vi "[ce] Find All Minima and Maxima of f(x).vi"(5 "accuracy":dbl=1e-08 format="%.2e", 6 "parameters":cluster{"name":string, "value":dbl}[](array[cluster]) {"value" format="%.2f"}, 7 "# points":u32=1000, 8 "error in":errorcluster, 9 "formula info":cluster{"formula":string, "x-variable":string}, 10 "end":dbl=1.0 format="%.2f", 11 "start":dbl format="%.2f") -> (0 "error out":errorcluster, 1 "ticks":u32, 2 "minima":cluster{"x":dbl[], "f(x)":dbl[]} {"f(x)" format="%.2f"; "x" format="%.2f"}, 3 "maxima":cluster{"x":dbl[], "f(x)":dbl[]} {"f(x)" format="%.2f"; "x" format="%.2f"})   [LabVIEW 2021]
doc: "The VI searches for all local minima and maxima of a 1D function in the specified interval. In addition, the VI allows specifying additional parameters and evaluating them in formula.\n\n::: CalcExpress Toolkit :::\nCopyright (c) 2000-2026 Konstantin Shifershteyn. All rights reserved."
panel:
  # "Example:\n\n accuracy: 1E-8 \n start: 0.0\n end: 1.0\n formula: x*x+sin(x)-1\n x-variable: x"
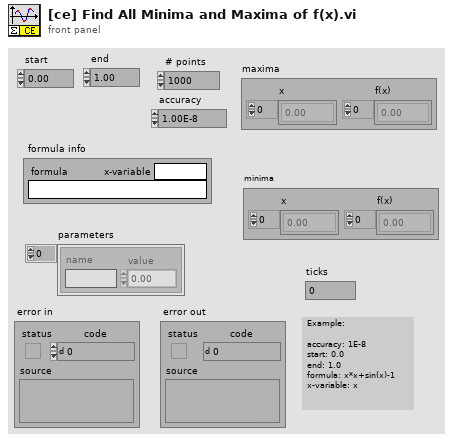
[diagram p1: front panel]
types:
  T1 = typedef "VarMan Variable Context Handle.ctl" = i32
  T2 = enum16{"create", "destroy", "set value", "get value"}
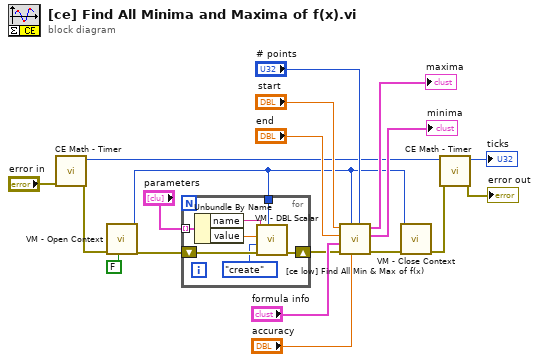
[diagram p0: block diagram]
diagram:
  n1 = call "CE Math - Timer.vi"("error in (no error)"="error in") -> ("error out"=w18:errorcluster, "ticks out"=w6:u32)  [unwired: 7 in]
  n2 = call "VM - Open Context.vi"("close loose contexts (F)"=FALSE ("close loose contexts (T)"), "error in"=w18) -> ("error out"=w4:errorcluster, "VC Handle out"=w2:T1)  [unwired: 7 in, 1 out]
  n3 = for {
    shift-right: [w23] -> w5
    shift-left: w4 -> [w24]
    tunnel: "parameters" -> [w21] mode=indexing
    tunnel: w2 -> [w20]
    n4 = Unbundle By Name(w21) -> ("name"=w25:string, "value"=w26:dbl)
    n5 = call "VM - DBL Scalar.vi"("VC Handle"=w20, "error in"=w24, "cmd"=T2."create", "value in"=w26, "name_spec"=w25) -> ("error out"=w23:errorcluster)  [unwired: 1 in, 5 out]
  }
  n6 = call "[ce low] Find All Min & Max of f(x).vi"("# points"="# points", "accuracy"="accuracy", "VC Handle"=w2, "error in"=w5, "formula info"="formula info", "end"="end", "start"="start") -> ("error out"=w17:errorcluster, "minima"=→"minima":cluster{"x":dbl[], "f(x)":dbl[]}, "maxima"=→"maxima":cluster{"x":dbl[], "f(x)":dbl[]})  [unwired: 2 in]
  n7 = call "VM - Close Context.vi"("error in"=w17, "VC Handle"=w2) -> ("error out"=w16:errorcluster)  [unwired: 8 in, 1 out]
  n8 = call "CE Math - Timer.vi"("error in (no error)"=w16, "ticks in"=w6) -> ("error out"=→"error out":errorcluster, "ticks out"=→"ticks":u32)  [unwired: 6 in]
